vi "Process Diff Images.vi"(7 "Debug? (F)":bool, 8 "error in (no error)":errorcluster, 11 "Report path":path) -> (0 "error out":errorcluster)   [LabVIEW 2021, in "Graphical Diff.lvlib"]
uses:
  Graphical Diff.lvlib
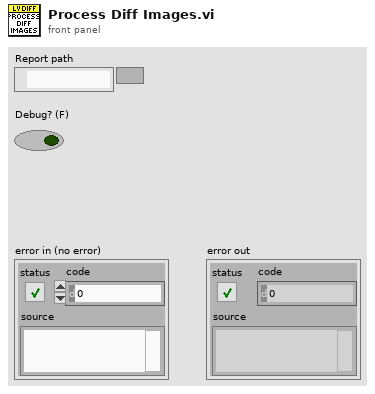
[diagram p1: front panel]
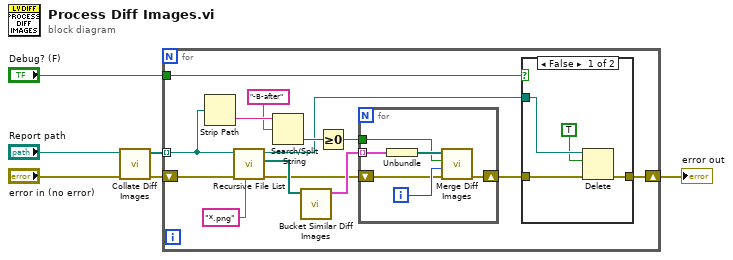
[diagram p0: block diagram]
diagram:
  n1 = call "Collate Diff Images.vi"("error in (no error)"="error in (no error)", "Report XML Path"="Report path") -> ("error out"=w5:errorcluster, "Collated Directories"=w2:path[])  [unwired: 8 in]
  n2 = for {
    shift-right: [w11] -> w6
    shift-left: w5 -> [w18]
    tunnel: w2 -> [w10] mode=indexing
    tunnel: "Debug? (F)" -> [w12]
    n3 = Strip Path(path=w10) -> (name=w16:string)  [unwired: 1 out]
    n4 = call <vilib>:"Recursive File List.vi"("pattern"="*.png", "error in (no error)"=w18, "Folder Path"=w10) -> ("error out"=w9:errorcluster, "All Files in Dir"=w20:path[], "dup Folder Path"=w7:path)  [unwired: 4 in, 2 out]
    n5 = Search/Split String(string=w16, search string/char (-)="-B-after" ("pattern")) -> (offset of match=w14:i32)  [unwired: 1 in, 2 out]
    n6 = call "Bucket Similar Diff Images.vi"("All PNG Files"=w20) -> ("All PNG Files (Bucketed by Near-Matches)"=w19:cluster{"Similar PNG Files":path[]}[])  [unwired: 9 in]
    n7 = Greater Or Equal To 0?(x=w14) -> (x >= 0?=w13:bool)
    n8 = for {
      tunnel: w19 -> [w31] mode=indexing
      tunnel: w13 -> [w29]
      shift-right: [w26] -> w8
      shift-left: w9 -> [w27]
      i -> [w28]
      n9 = Unbundle(w31) -> ("Similar PNG Files"=w30:path[])
      n10 = call "Merge Diff Images.vi"("error in (no error)"=w27, "ID"=w28, "Before = F | After = T?"=w29, "Diff PNG Files"=w30) -> ("error out"=w26:errorcluster)  [unwired: 6 in]
    }
    n11 = case shown="False" w12 {
      tunnel: [w24 w25] -> w11
      tunnel: w7 -> [w23 _]
      tunnel: w8 -> [w21 w25]
      frame False {
        n12 = Delete(path (use dialog)=w23, entire hierarchy (F)=TRUE, error in=w21) -> (error out=w24:errorcluster)  [unwired: 2 in, 2 out]
      }
      frame True {
        # "leave collated dirs present if debugging"
      }
    }
  }
  "error out" <- w6
